vi "PAQ_getPointers.vi"(7 "Layer":i32, 8 "error in (no error)":errorcluster, 11 "FAMM in":refnum<class "FAMM.lvclass">) -> (0 "error out":errorcluster, 1 "Pointers":cluster{"Pointer":i32, "Carry":i32}, 3 "FAMM out":refnum<class "FAMM.lvclass">)   [LabVIEW 2020]
doc: "Get PAQ memory layer pointers"
uses:
  FAMM.lvclass
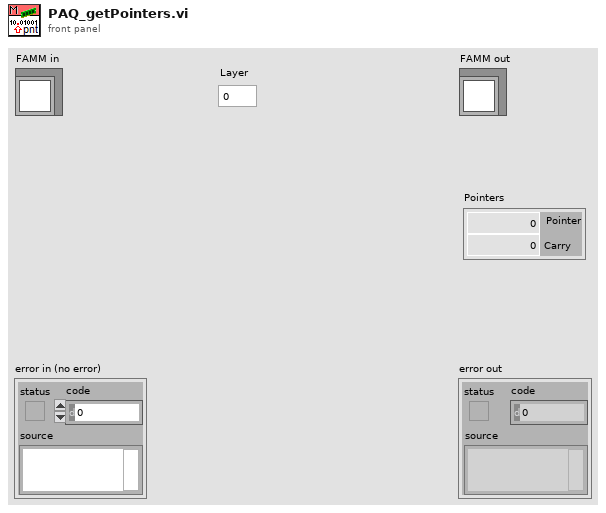
[diagram p1: front panel]
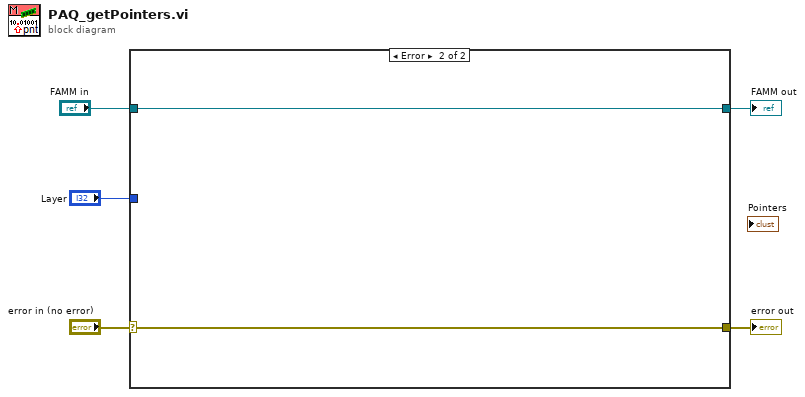
[diagram p0: block diagram]
diagram:
  n1 = case shown="Error" "error in (no error)" {
    selector: "error in (no error)" -> [w6 w9]
    tunnel: [w6 w9] -> w4
    tunnel: [w7 w8] -> w2
    tunnel: "FAMM in" -> [w7 w8]
    tunnel: "Layer" -> [_ _]
    frame No Error {
    }
    frame Error {
    }
  }
  "error out" <- w4
  "FAMM out" <- w2
